vi "Get VI Library Path.vi"() -> (2 "VI Library":path)   [LabVIEW 2020, in "Paths.lvlib"]
doc: "Returns the vi.lib folder that this copy of LUnit is installed in, found by walking up from this VI's own path to the nearest folder named vi.lib. Works for a regular install into the LabVIEW folder, an LVAddon and an lvpm virtual environment. Falls back to LabVIEW's native VI Library path if no vi.lib folder is found (e.g. when running from source). Use this instead of the VI Library constant for any path to LUnit's own files; siblings such as resource and project are found with ..\\resource etc. relative to the returned path."
uses:
  Paths.lvlib
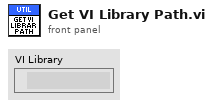
[diagram p1: front panel]
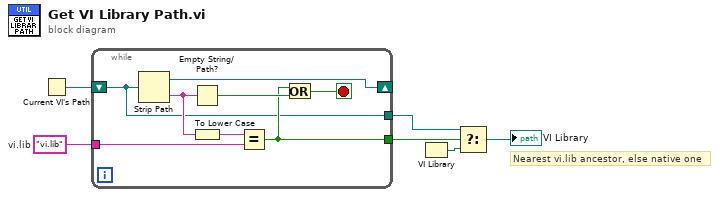
[diagram p0: block diagram]
diagram:
  w6 = "vi.lib"  # vi.lib
  # "Nearest vi.lib ancestor, else native one"
  n1 = Current VI's Path() -> (path=w5:path)
  n2 = while {
    tunnel: w6 -> [w12]
    shift-right: [w14] -> _
    shift-left: w5 -> [w7]
    tunnel: [w8] -> w3
    tunnel: [w7] -> w4
    stop <- w9 stop-if-true
    n3 = Strip Path(path=w7) -> (stripped path=w14:path, name=w11:string)
    n4 = Empty String/Path?(string/path=w11) -> (empty?=w10:bool)
    n5 = To Lower Case(string=w11) -> (all lower case string=w13:string)
    n6 = Equal?(x=w13, y=w12) -> (x = y?=w8:bool)
    n7 = Or(x=w8, y=w10) -> (x .or. y?=w9:bool)
  }
  n8 = VI Library() -> (path=w2:path)
  n9 = Select(t=w4, s=w3, f=w2) -> (s? t:f=→"VI Library":path)
